vi "Script.vi"(8 "error in":errorcluster, 11 "Msg in":refnum<class "Msg.lvclass">) -> (0 "error out":errorcluster, 3 "Msg out":refnum<class "Msg.lvclass">)   [LabVIEW 2020, in "_Rescript.lvlib" / "Msg.lvlib" / "Msg.lvclass"]
uses:
  Msg.lvclass
  Msg.lvclass/Msg.ctl
  IO.ctl
  Script PD.vi
  Script Con And Wire.vi
  Script BunUnbun IO Wire.vi
  Duplicate Control To FP.vi
  Terminal Attributes Descending Order.vi
  Find Pane.vi
  SubVI Terminals.vi
  <vilib>/Utility/traverseref.llb/TRef Find Object By Label.vi
  Script Control To ConPane.vi
  _Shared/Name Specs/Name Specs.lvclass
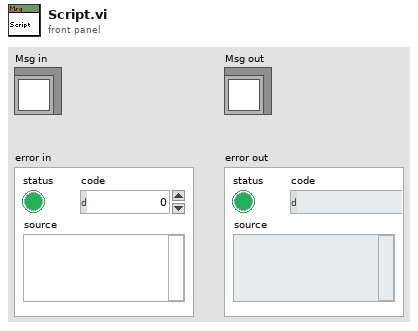
[diagram p1: front panel]
types:
  T1 = typedef "_Rescript.lvlib/Msg.lvlib/Msg.lvclass/IO.ctl" = enum16{"Input", "Output"}
  T2 = typedef "_Rescript.lvlib/Msg.lvlib/Msg.lvclass/Name Msg IO.ctl" = cluster{"PD Control (Class)":refnum<vi>, "PD Cluster (Class)":refnum<vi>, "Init Msg IO VI (Class)":refnum<vi>, "Read Msg IO VI (Class)":refnum<vi>, "Init Msg IO VI (Lib)":refnum<vi>, "Read Msg IO VI (Lib)":refnum<vi>, "Terminal Attributes (Init)":T3, "Terminal Attributes (Read)":T3}
  T3 = typedef "_Rescript.lvlib/Terminal Attributes.ctl" = map{i32, T4}
  T4 = typedef "_Rescript.lvlib/Attributes.ctl" = cluster{"Control":refnum<vi>, "Wire Rule":enum16{"Invalid Wire Rule", "Required", "Recommended", "Optional", "Dynamic Dispatch"}}
  T5 = typedef "_Shared.lvlib/Name Stuff.ctl" = cluster{"Type (Enum)":T6, "Type (String)":string, "Name Library File Path":path, "Name":string, "Name Type":string}
  T6 = typedef "_Shared.lvlib/Type.ctl" = enum16{"Actor", "Msg"}
  T7 = typedef "_Rescript.lvlib/Msg.lvlib/Msg.lvclass/Name Msg.ctl" = cluster{"Execute VI (Class)":refnum<vi>}
  T8 = typedef "_Rescript.lvlib/Msg.lvlib/Msg.lvclass/Name.ctl" = cluster{"Name VI (Lib)":refnum<vi>, "Init Msg VI (Lib)":refnum<vi>, "Call VI (Lib)":refnum<vi>, "Recurse VI (Lib)":refnum<vi>, "Tell Self VI (Lib)":refnum<vi>, "Tell Parent VI (Lib)":refnum<vi>, "Tell Child VI (Lib)":refnum<vi>, "Tell Reply VI (Lib)":refnum<vi>}
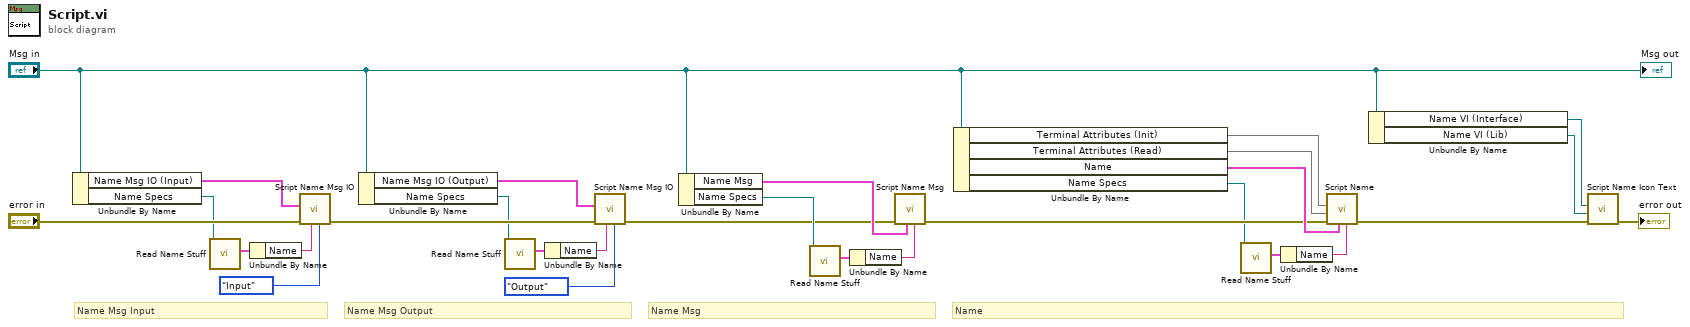
[diagram p0: block diagram]
diagram:
  # "Name"
  # "Name Msg"
  # "Name Msg Output"
  # "Name Msg Input"
  n1 = Unbundle By Name("Msg in") -> ("Name Msg IO (Input)"=w9:T2, "Name Specs"=w2:refnum<class "Name Specs.lvclass">)
  n2 = call "Read Name Stuff.vi"("Name Specs in"=w2) -> ("Name Stuff"=w5:T5)  [unwired: 10 in]
  n3 = Unbundle By Name(w5) -> ("Name"=w4:string)
  n4 = call "Script Name Msg IO.vi"("IO"=IO."Input", "Name"=w4, "error in"="error in", "Name Msg IO"=w9) -> ("error out"=w10:errorcluster)  [unwired: 7 in]
  n5 = Unbundle By Name("Msg in") -> ("Name Msg IO (Output)"=w12:T2, "Name Specs"=w1:refnum<class "Name Specs.lvclass">)
  n6 = call "Read Name Stuff.vi"("Name Specs in"=w1) -> ("Name Stuff"=w6:T5)  [unwired: 10 in]
  n7 = Unbundle By Name(w6) -> ("Name"=w3:string)
  n8 = call "Script Name Msg IO.vi"("IO"=IO."Output", "Name"=w3, "error in"=w10, "Name Msg IO"=w12) -> ("error out"=w14:errorcluster)  [unwired: 7 in]
  n9 = Unbundle By Name("Msg in") -> ("Name Msg"=w18:T7, "Name Specs"=w19:refnum<class "Name Specs.lvclass">)
  n10 = call "Read Name Stuff.vi"("Name Specs in"=w19) -> ("Name Stuff"=w22:T5)  [unwired: 10 in]
  n11 = Unbundle By Name(w22) -> ("Name"=w21:string)
  n12 = call "Script Name Msg.vi"("Name"=w21, "Name Msg"=w18, "error in"=w14) -> ("error out"=w20:errorcluster)  [unwired: 8 in]
  n13 = Unbundle By Name("Msg in") -> ("Terminal Attributes (Init)"=w25:T3, "Terminal Attributes (Read)"=w24:T3, "Name"=w23:T8, "Name Specs"=w16:refnum<class "Name Specs.lvclass">)
  n14 = call "Read Name Stuff.vi"("Name Specs in"=w16) -> ("Name Stuff"=w17:T5)  [unwired: 10 in]
  n15 = Unbundle By Name(w17) -> ("Name"=w15:string)
  n16 = call "Script Name.vi"(4:"Name"=w15, 6:"Name"=w23, "error in"=w20, "Name Msg IO (Output).Terminal Attributes (Read)"=w24, "Name Msg IO (Input).Terminal Attributes (Init)"=w25) -> ("error out"=w26:errorcluster)  [unwired: 6 in]
  n17 = Unbundle By Name("Msg in") -> ("Name VI (Interface)"=w28:refnum<vi>, "Name VI (Lib)"=w27:refnum<vi>)
  n18 = call "Script Name Icon Text.vi"("error in"=w26, "Name.Name VI (Lib)"=w27, "Name jettl Msg.Name VI (Interface)"=w28) -> ("error out"=→"error out":errorcluster)  [unwired: 8 in]
  "Msg out" <- "Msg in"
